vi "Constructor.vi"(6 "Database_location":path=path "D:/Sgraph_database", 8 "error in (no error)":errorcluster, 9 "File extention":string, 10 "DatabaseType":string, 11 "DBAL in":refnum<class "DBAL.lvclass">) -> (0 "error out":errorcluster, 2 "DBAL_class":refnum<data-value>, 3 "DBAL out":refnum<class "DBAL.lvclass">)   [LabVIEW 2020, in "Sgraph_lib_V1.lvlib" / "DBAL.lvclass"]
doc: "The DBAL constructor will make the first DBAL class instance depending on the required database type as defined in the historian ini file."
uses:
  DBAL.lvclass
  DBAL-BIN.lvclass
  C:/Sgraph/Sgraph/source/DBAL/DBAL.lvclass
  DBAL-BIN.lvclass/DBAL-BIN.ctl
  DBAL-SQLite.lvclass
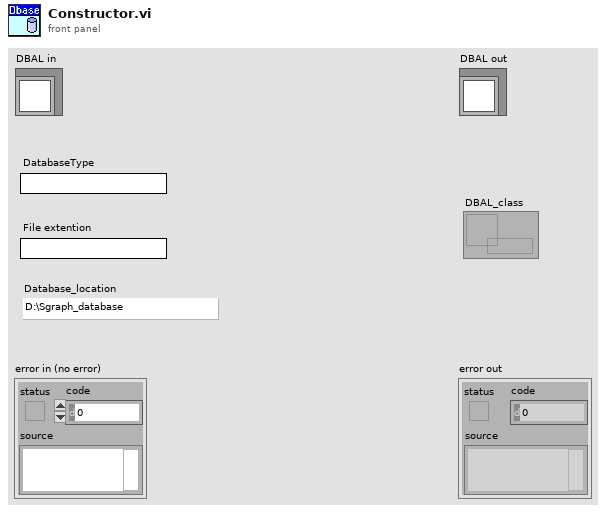
[diagram p1: front panel]
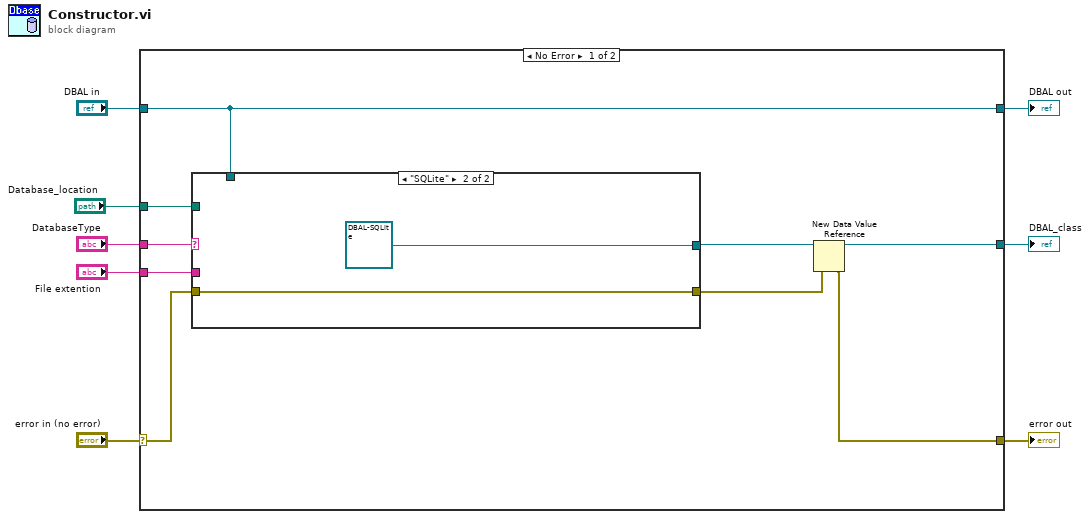
[diagram p0: block diagram]
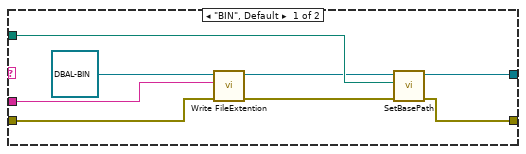
[diagram p2: hidden frame]
diagram:
  n1 = case shown="No Error" "error in (no error)" {
    selector: "error in (no error)" -> [w14 w29]
    tunnel: [w16 w29] -> w7
    tunnel: [w10 w28] -> w5
    tunnel: "DBAL in" -> [w10 w28]
    tunnel: "DatabaseType" -> [w17 _]
    tunnel: [w15 _] -> w3
    tunnel: "File extention" -> [w12 _]
    tunnel: "Database_location" -> [w11 _]
    frame No Error {
      n2 = case shown="\"SQLite\"" w17 {
        tunnel: [w22 refnum<class "DBAL-SQLite.lvclass"> refnum ("DBAL-SQLite.lvclass")] -> w9
        tunnel: w10 -> [_ _]
        tunnel: w14 -> [w24 w26]
        tunnel: [w20 w26] -> w13
        tunnel: w12 -> [w23 _]
        tunnel: w11 -> [w19 _]
        frame "BIN", Default {
          n3 = call "Write FileExtention.vi"("error in (no error)"=w24, "FileExtention"=w23, "DBAL-BIN in"=refnum<class "DBAL-BIN.lvclass"> refnum ("DBAL-BIN.lvclass")) -> ("error out"=w21:errorcluster, "DBAL-BIN out"=w18:refnum<class "DBAL-BIN.lvclass">)  [unwired: 7 in]
          n4 = call "SetBasePath.vi"("error in (no error)"=w21, "base_path"=w19, "DBAL-BIN in"=w18) -> ("error out"=w20:errorcluster, "DBAL-BIN out"=w22:refnum<class "DBAL-BIN.lvclass">)  [unwired: 7 in]
        }
        frame "SQLite" {
        }
      }
      n5 = New Data Value Reference(data value=w9, error in=w13) -> (data value reference=w15:refnum<data-value>, error out=w16:errorcluster)
    }
    frame Error {
    }
  }
  "error out" <- w7
  "DBAL out" <- w5
  "DBAL_class" <- w3
